vi "Read Batch Buffer.vi"(8 "error in (no error)":errorcluster, 11 "OD Batch in":refnum<class "OD Batch.lvclass">) -> (0 "error out":errorcluster, 2 "Batch Buffer":u8[](array[numeric]), 3 "OD Batch out":refnum<class "OD Batch.lvclass">)   [LabVIEW 2023, in "xnet_canopen.lvlib" / "OD Batch.lvclass"]
uses:
  OD Batch.lvclass
  OD Batch.lvclass/OD Batch.ctl
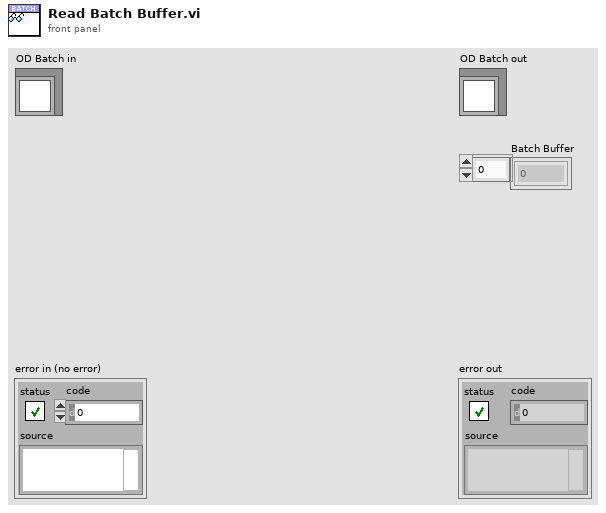
[diagram p1: front panel]
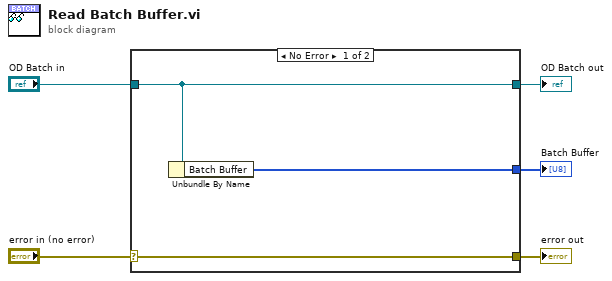
[diagram p0: block diagram]
diagram:
  n1 = case shown="No Error" "error in (no error)" {
    selector: "error in (no error)" -> [w8 w9]
    tunnel: [w8 w9] -> w4
    tunnel: [w7 w10] -> w2
    tunnel: "OD Batch in" -> [w7 w10]
    tunnel: [w6 _] -> w1
    frame No Error {
      n2 = Unbundle By Name(w7) -> ("Batch Buffer"=w6:u8[])
    }
    frame Error {
    }
  }
  "error out" <- w4
  "OD Batch out" <- w2
  "Batch Buffer" <- w1
